vi "Init.vi"(8 "error in (no error)":errorcluster, 10 "Instrument String":variant, 11 "NI Scope in":refnum<class "NI Scope.lvclass">) -> (0 "error out":errorcluster, 2 "Found?":bool=TRUE, 3 "NI Scope out":refnum<class "NI Scope.lvclass">)   [LabVIEW 2025, in "Scope.lvlib" / "NI Scope.lvclass"]
uses:
  NI Scope.lvclass
  Scope configuration/Scope configuration.lvclass
  NI Scope.lvclass/NI Scope.ctl
  Users/Public/Documents/Sandia National Labs/TSS Plugin/Abstract Engine.lvlibp/Instrument configuration/Read Instrument Setting.vi
  Users/Public/Documents/Sandia National Labs/TSS Plugin/CEF.lvlibp/serializable configuration/CEF_serializable configuration.lvclass
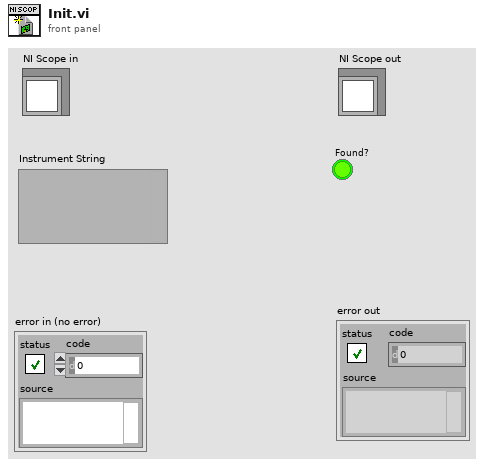
[diagram p1: front panel]
types:
  T1 = typedef "Abstract Engine.lvlibp/Instrument configuration.lvclass/Default Instrument.ctl" = cluster{"Type":string, "Address":string, "SW Alias":string, "Description":string, "Enabled":bool}
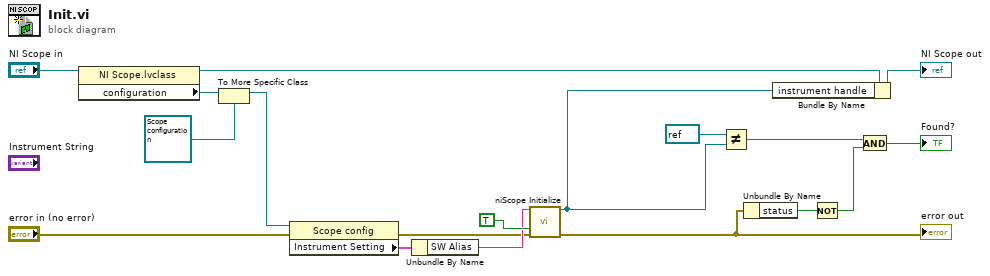
[diagram p0: block diagram]
diagram:
  n1 = property class="NI Scope.lvclass"(reference="NI Scope in") -> (reference out=w1:refnum<class "NI Scope.lvclass">, "configuration"=w12:refnum<class "CEF_serializable configuration.lvclass">)  [unwired: 1 in, 1 out]
  n2 = To More Specific Class(target class=refnum<class "Scope configuration.lvclass"> refnum ("Scope.lvlib:Scope configuration.lvclass"), reference=w12) -> (specific class reference=w11:refnum<class "Scope configuration.lvclass">)  [unwired: 1 in, 1 out]
  n3 = property class="Scope config"(reference=w11, error in="error in (no error)") -> (error out=w4:errorcluster, "Instrument Setting"=w13:T1)  [unwired: 1 out]
  n4 = Unbundle By Name(w13) -> ("SW Alias"=w15:string)
  n5 = call <instrlib>:"niScope Initialize.vi"("resource name"=w15, "reset device"=TRUE, "error in"=w4) -> ("instrument handle"=w3:refnum<k15>, "error out"=w2:errorcluster)  [unwired: 11 in]
  "error out" <- w2
  n6 = Not Equal?(x=refnum<k15> refnum, y=w3) -> (x != y?=w9:bool)
  n7 = Unbundle By Name(w2) -> ("status"=w8:bool)
  n8 = Bundle By Name(cluster=w1, "instrument handle"=w3) -> (→"NI Scope out":refnum<class "NI Scope.lvclass">)
  n9 = Not(x=w8) -> (.not. x?=w6:bool)
  n10 = And(x=w9, y=w6) -> (x .and. y?=→"Found?":bool)
